vi "RemoteVI Check Parse Input.vi"() -> (4 "labels":string[](array[string]), 6 "expected":string[](array[string]), 8 "actual":string[](array[string]), 10 "failures":i32)   [LabVIEW 2020]
doc: "Test support, generated by tests/caraya/build.py from tests/vectors/input.json - do not edit. Calls RemoteVI Parse Input.vi once per vector: a null result is kind invalid; the other outputs are compared only where the vector's result names them (mouse: msg x y wParam, key: msg wParam lParam, ack: seq, close: id, splitter: id and x as pos). Outputs, one element per vector: labels (the vector's name), expected (rendered from the vector), actual (the VI's result rendered the same way), and failures, the number of vectors whose expected and actual differ."
uses:
  source/RemoteVI.lvlib
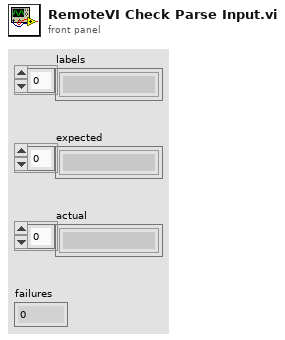
[diagram p1: front panel]
types:
  T1 = cluster{"name":string, "text":string, "expect":string}[]
  T2 = enum16{"invalid", "mouse", "key", "ack", "close", "splitter"}
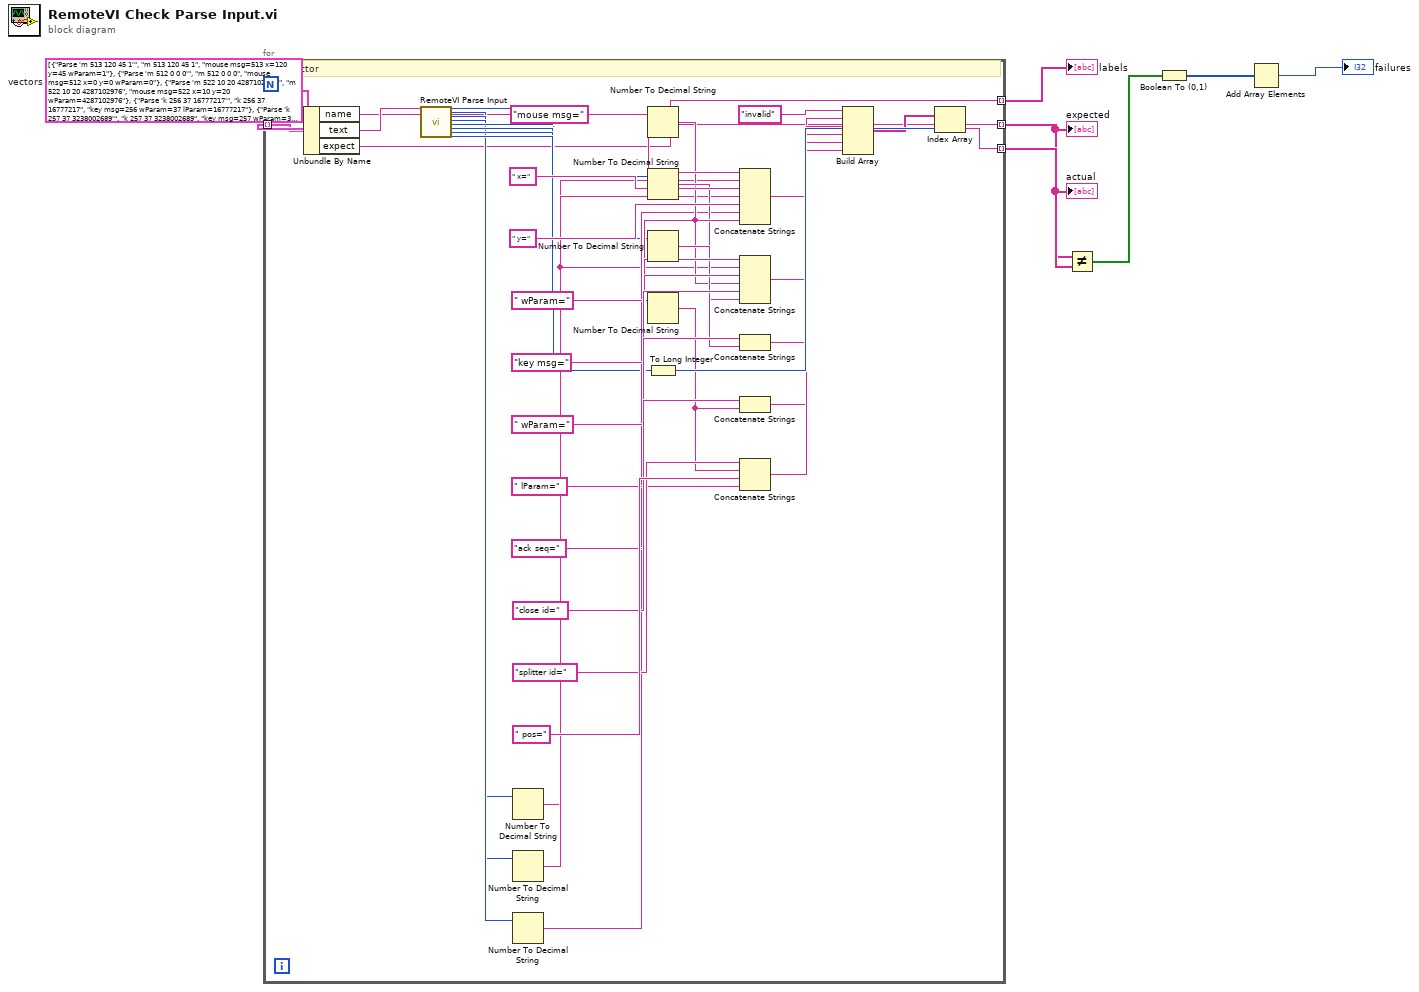
[diagram p0: block diagram]
diagram:
  w1 = T1 [{"name"="Parse 'm 513 120 45 1'", "text"="m 513 120 45 1", "expect"="mouse msg=513 x=120 y=45 wParam=1"}, {"name"="Parse 'm 512 0 0 0'", "text"="m 512 0 0 0", "expect"="mouse msg=512 x=0 y=0 wParam=0"}, {"name"="Parse 'm 522 10 20 4287102976'", "text"="m 522 10 20 4287102976", "expect"="mouse msg=522 x=10 y=20 wParam=4287102976"}, {"name"="Parse 'k 256 37 16777217'", "text"="k 256 37 16777217", "expect"="key msg=256 wParam=37 lParam=16777217"}, {"name"="Parse 'k 257 37 3238002689'", "text"="k 257 37 3238002689", "expect"="key msg=257 wParam=37 lParam=3238002689"}, {"name"="Parse 'k 258 65 1'", "text"="k 258 65 1", "expect"="key msg=258 wParam=65 lParam=1"}, {"name"="Parse 'a 12'", "text"="a 12", "expect"="ack seq=12"}, {"name"="Parse 'a'", "text"="a", "expect"="invalid"}, {"name"="Parse 'm 513 1 2'", "text"="m 513 1 2", "expect"="invalid"}, {"name"="Parse 'x 1 2 3'", "text"="x 1 2 3", "expect"="invalid"}, {"name"="Parse 'm 513 a b c'", "text"="m 513 a b c", "expect"="invalid"}, {"name"="Parse ''", "text"="", "expect"="invalid"}, {"name"="Parse 'm 513 1.5 2 0'", "text"="m 513 1.5 2 0", "expect"="invalid"}, {"name"="Parse 'x 5113012'", "text"="x 5113012", "expect"="close id=5113012"}, {"name"="Parse 'x'", "text"="x", "expect"="invalid"}, {"name"="Parse 'x -1'", "text"="x -1", "expect"="invalid"}, {"name"="Parse 'x 1 2'", "text"="x 1 2", "expect"="invalid"}, {"name"="Parse 'a '", "text"="a ", "expect"="invalid"}, {"name"="Parse 'a  12'", "text"="a  12", "expect"="invalid"}, {"name"="Parse 'a 12 '", "text"="a 12 ", "expect"="invalid"}, {"name"="Parse 'a 4294967295'", "text"="a 4294967295", "expect"="ack seq=4294967295"}, {"name"="Parse 'a 4294967296'", "text"="a 4294967296", "expect"="invalid"}, {"name"="Parse 'k 256 -2147483648 0'", "text"="k 256 -2147483648 0", "expect"="key msg=256 wParam=18446744071562067968 lParam=0"}, {"name"="Parse 'k 256 -2147483649 0'", "text"="k 256 -2147483649 0", "expect"="invalid"}, {"name"="Parse 'a 1x'", "text"="a 1x", "expect"="invalid"}, {"name"="Parse 'a -'", "text"="a -", "expect"="invalid"}, {"name"="Parse 'a 1e3'", "text"="a 1e3", "expect"="invalid"}, {"name"="Parse 's 0 300'", "text"="s 0 300", "expect"="splitter id=0 pos=300"}, {"name"="Parse 's 1 -12'", "text"="s 1 -12", "expect"="splitter id=1 pos=-12"}, {"name"="Parse 's 2'", "text"="s 2", "expect"="invalid"}, {"name"="Parse 's -1 5'", "text"="s -1 5", "expect"="invalid"}, {"name"="Parse 's 0 5 6'", "text"="s 0 5 6", "expect"="invalid"}]  # vectors
  n1 = for {
    tunnel: w1 -> [w8] mode=indexing
    tunnel: [w9] -> w2 mode=indexing
    tunnel: [w11] -> w3 mode=indexing
    tunnel: [w46] -> w4 mode=indexing
    # "One vector"
    n2 = Unbundle By Name(w8) -> ("name"=w9:string, "text"=w10:string, "expect"=w11:string)
    n3 = call "RemoteVI Parse Input.vi"("text"=w10) -> ("kind"=w12:T2, "msg"=w13:u32, "x"=w14:i32, "y"=w15:i32, "wParam"=w16:u64, "lParam"=w17:i64, "seq"=w18:u32, "id"=w19:u64)  [unwired: 19 in]
    n4 = Number To Decimal String(number=w13) -> (decimal integer string=w20:string)  [unwired: 1 in]
    n5 = Number To Decimal String(number=w14) -> (decimal integer string=w21:string)  [unwired: 1 in]
    n6 = Number To Decimal String(number=w15) -> (decimal integer string=w22:string)  [unwired: 1 in]
    n7 = Number To Decimal String(number=w16) -> (decimal integer string=w23:string)  [unwired: 1 in]
    n8 = Number To Decimal String(number=w17) -> (decimal integer string=w24:string)  [unwired: 1 in]
    n9 = Number To Decimal String(number=w18) -> (decimal integer string=w25:string)  [unwired: 1 in]
    n10 = Number To Decimal String(number=w19) -> (decimal integer string=w26:string)  [unwired: 1 in]
    n11 = To Long Integer(number=w12) -> (32bit integer=w45:i32)
    n12 = Concatenate Strings("mouse msg=", w20, " x=", w21, " y=", w22, " wParam=", w23) -> (w31:string)
    n13 = Concatenate Strings("key msg=", w20, " wParam=", w23, " lParam=", w24) -> (w35:string)
    n14 = Concatenate Strings("ack seq=", w25) -> (w37:string)
    n15 = Concatenate Strings("close id=", w26) -> (w39:string)
    n16 = Concatenate Strings("splitter id=", w26, " pos=", w21) -> (w42:string)
    n17 = Build Array("invalid", w31, w35, w37, w39, w42) -> (w44:string[])
    n18 = Index Array(array=w44, index=w45) -> (element=w46:string)
  }
  "labels" <- w2
  "expected" <- w3
  "actual" <- w4
  n19 = Not Equal?(x=w3, y=w4) -> (x != y?=w5:bool[])
  n20 = Boolean To (0,1)(Boolean=w5) -> (0, 1=w6:i16[])
  n21 = Add Array Elements(numeric array=w6) -> (sum=→"failures":i16)
